vi "Write User Data.vi"(8 "error in (no error)":errorcluster, 10 "User Data":T1, 11 "user Data Path":path) -> (0 "error out":errorcluster)   [LabVIEW 2018]
doc: "Writes the user data to the configuration file specified by user <b>Data Path</b>. Creates or replaces the file, opens the configuration file, writes the contents of the User Data input and closes the file reference. Propagates any errors through the error cluster."
uses:
  <vilib>/TABOADA/Config Files Management/Config Files Management/config data--cluster.ctl
  <vilib>/TABOADA/Config Files Management/Config Files Management/Config Files Management.lvlib
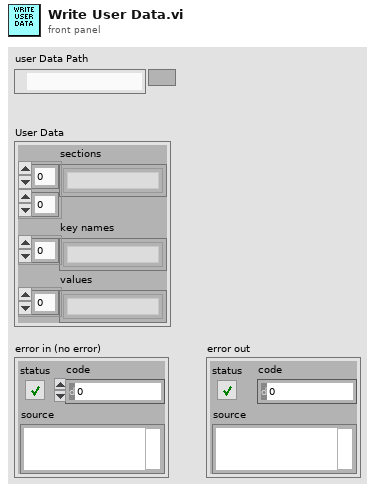
[diagram p1: front panel]
types:
  T1 = typedef "Config Files Management.lvlib/config data--cluster.ctl" = cluster{"sections":string[][], "key names":string[], "values":string[]}
  T2 = enum16{"open", "replace", "create", "open or create", "replace or create", "replace or create with confirmation"}
  T3 = typedef "NI_LVConfig.lvlib/Config Data RefNum.ctl" = refnum<k1>
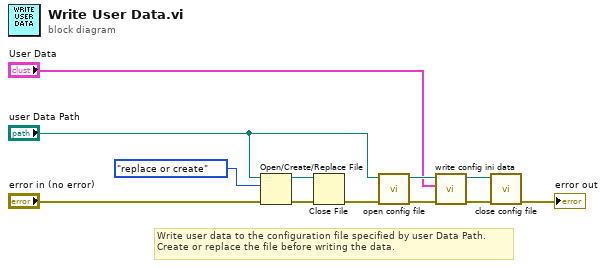
[diagram p0: block diagram]
diagram:
  # "Write user data to the configuration file specified by user Data Path.\nCreate or replace the file before writing the data."
  n1 = Open/Create/Replace File(file path (use dialog)="user Data Path", error in="error in (no error)", operation (0:open)=T2."replace or create") -> (refnum out=w8:refnum<file>, error out=w9:errorcluster)  [unwired: 3 in, 1 out]
  n2 = Close File(refnum=w8, error in=w9) -> (error out=w12:errorcluster)  [unwired: 1 out]
  n3 = call <vilib>:"open config file.vi"("error in (no error)"=w12, "configuration file path"="user Data Path") -> ("error out"=w10:errorcluster, "Refnum out"=w11:T3)  [unwired: 7 in, 1 out]
  n4 = call <vilib>:"write config ini data.vi"("error in (no error)"=w10, "data in"="User Data", "Refnum in"=w11) -> ("error out"=w4:errorcluster, "Refnum out"=w5:T3)  [unwired: 7 in]
  n5 = call <vilib>:"close config file.vi"("error in (no error)"=w4, "Refnum in"=w5) -> ("error out"=→"error out":errorcluster)  [unwired: 9 in]
